vi "add data.vi"(10 "nombre":string) -> (2 "New Data":string[](array[string]))   [LabVIEW 2021]
panel:
  in  "Accept":bool
  in  "Service":string
  in  "frais":string
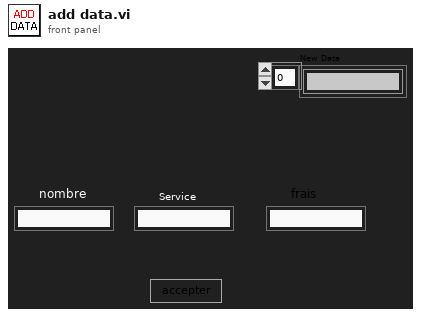
[diagram p1: front panel]
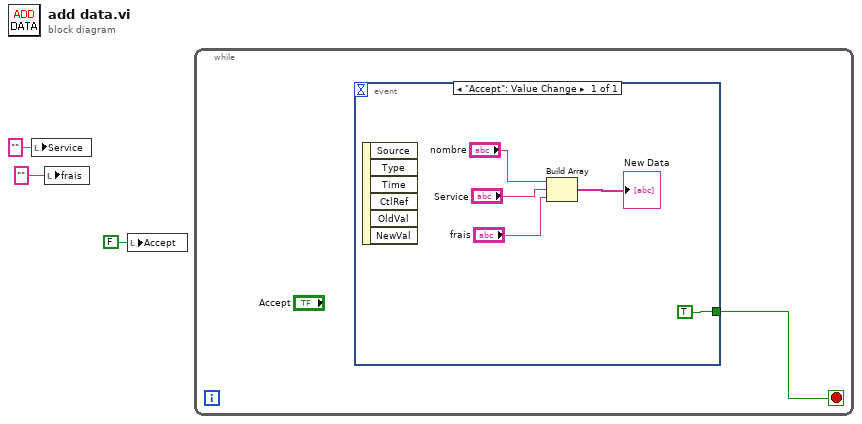
[diagram p0: block diagram]
diagram:
  n1 = local write "Service"("" ("Service")) -> ()
  n2 = local write "frais"("" ("charge")) -> ()
  n3 = local write "Accept"(FALSE ("Accept")) -> ()
  n4 = while {
    stop <- w4 stop-if-true
    n5 = event shown="[0] \"Accept\": Value Change" {
      selector: _ -> [_]
      dyn-events: _ -> [_]
      timeout: _ -> [_]
      tunnel: [TRUE] -> w4
      event "Accept": Value Change {
        n6 = event-data() -> ()  [unwired: 1 in, 6 out]
        n7 = Build Array("nombre", "Service", "frais") -> (→"New Data":string[])
      }
    }
  }
